vi "Read Projects.vi"(8 "error in (no error)":errorcluster, 11 "Project Store in":refnum<class "Project Store.lvclass">) -> (0 "error out":errorcluster, 2 "Project List":T1, 3 "Project Store out":refnum<class "Project Store.lvclass">)   [LabVIEW 2024, in "Project Store.lvclass"]
doc: "Reads one field of this class's private data. Generated by lvai_create_accessors from the class private data control."
uses:
  Project Store.lvclass
  Project Store.lvclass/Project Store.ctl
  Rows/Project.ctl
  Rows/Project List.ctl
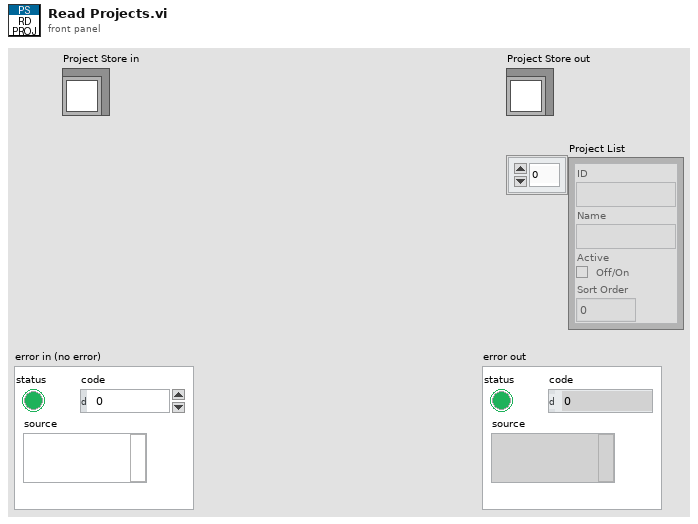
[diagram p1: front panel]
types:
  T1 = typedef "Project List.ctl" = T2[]
  T2 = typedef "Project.ctl" = cluster{"ID":string, "Name":string, "Active":bool, "Sort Order":i32}
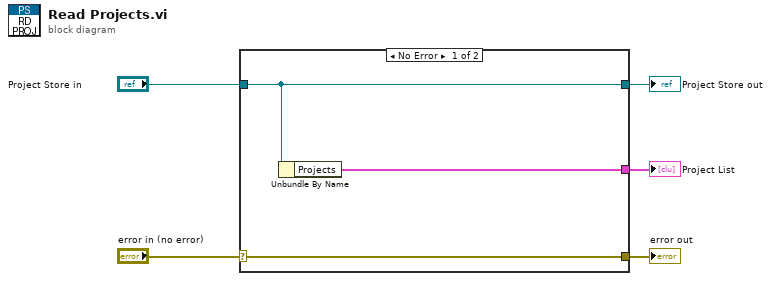
[diagram p0: block diagram]
diagram:
  n1 = case shown="No Error" "error in (no error)" {
    selector: "error in (no error)" -> [w8 w9]
    tunnel: [w8 w9] -> w4
    tunnel: [w7 w10] -> w2
    tunnel: "Project Store in" -> [w7 w10]
    tunnel: [w6 _] -> w1
    frame No Error {
      n2 = Unbundle By Name(w7) -> ("Projects"=w6:T1)
    }
    frame Error {
    }
  }
  "error out" <- w4
  "Project Store out" <- w2
  "Project List" <- w1
